vi "VHistFile - Tag to file name.vi"(4 "file tag":string) -> (1 "file name":string)   [LabVIEW 2021]
doc: "::: CalcExpress Toolkit :::\nCopyright (c) 2000-2026 Konstantin Shifershteyn. All rights reserved."
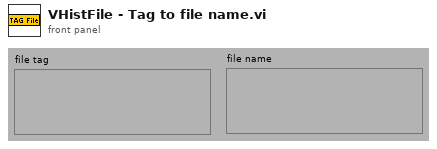
[diagram p1: front panel]
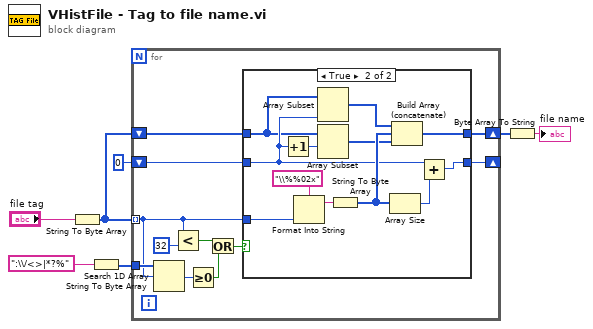
[diagram p0: block diagram]
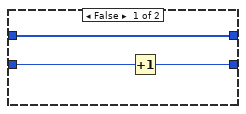
[diagram p2: hidden frame]
diagram:
  n1 = String To Byte Array(string="file tag") -> (unsigned byte array=w6:u8[])
  n2 = String To Byte Array(string=":\\/<>|*?%") -> (unsigned byte array=w1:u8[])
  n3 = for {
    tunnel: w6 -> [w8] mode=indexing
    tunnel: w1 -> [w17]
    shift-right: [w11] -> w4
    shift-left: w6 -> [w12]
    shift-right: [w9] -> _
    shift-left: 0 -> [w10]
    n4 = Search 1D Array(1D array=w17, element=w8) -> (index of element=w16:i32)  [unwired: 1 in]
    n5 = Less?(x=w8, y=u8 32) -> (x < y?=w14:bool)
    n6 = Greater Or Equal To 0?(x=w16) -> (x >= 0?=w13:bool)
    n7 = Or(x=w14, y=w13) -> (x .or. y?=w15:bool)
    n8 = case shown="True" w15 {
      tunnel: w12 -> [w21 w22]
      tunnel: [w21 w28] -> w11
      tunnel: w10 -> [w20 w24]
      tunnel: [w19 w29] -> w9
      tunnel: w8 -> [_ w32]
      frame False {
        n9 = Increment(x=w20) -> (x+1=w19:i32)
      }
      frame True {
        n10 = Increment(x=w24) -> (x+1=w27:i32)
        n11 = Format Into String(format string="\\%%02x", w32) -> (resulting string=w31:string)  [unwired: 2 in, 1 out]
        n12 = Array Subset(array=w22, length=w24) -> (w25:u8[])  [unwired: 1 in]
        n13 = Array Subset(array=w22, index=w27) -> (w26:u8[])  [unwired: 1 in]
        n14 = String To Byte Array(string=w31) -> (unsigned byte array=w30:u8[])
        n15 = Array Size(array=w30) -> (size(s)=w23:i32)
        n16 = Build Array (concatenate)(w25, w30, w26) -> (w28:u8[])
        n17 = Add(x=w24, y=w23) -> (x+y=w29:i32)
      }
    }
  }
  n18 = Byte Array To String(unsigned byte array=w4) -> (string=→"file name":string)
